vi "query Marker Frequency Count Value.vi"(8 "error in (no error)":errorcluster, 10 "Marker Index":i32=1 min=1, 11 "FSV-40N in":refnum<class "FSV-40N.lvclass">) -> (0 "error out":errorcluster, 2 "Marker Value":T1 {"X-axis" format="%#_6p"}, 3 "FSV-40N out":refnum<class "FSV-40N.lvclass">)   [LabVIEW 2023, in "Spectrum Analyzer.lvlib" / "FSV-40N.lvclass"]
uses:
  FSV-40N.lvclass
  FSV-40N.lvclass/FSV-40N.ctl
  TYPE DEFINITION/TYPE Marker Control Mode.ctl
  Spectrum Analyzer.lvlib
  <vilib>/ErrorRing/Error Ring.xnode
  TYPE DEFINITION/TYPE Marker Value.ctl
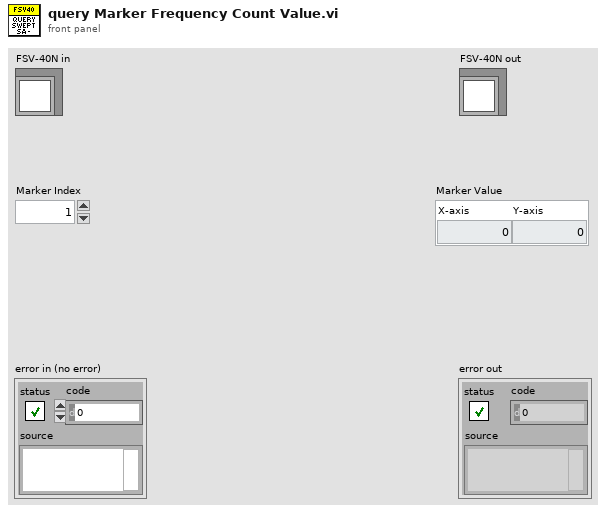
[diagram p1: front panel]
types:
  T1 = typedef "Spectrum Analyzer.lvlib/TYPE Marker Value.ctl" = cluster{"X-axis":dbl, "Y-axis":dbl}
  T2 = typedef "Spectrum Analyzer.lvlib/TYPE Marker Control Mode.ctl" = enum16{"Normal", "Delta", "Off"}
  T3 = typedef "Spectrum Analyzer.lvlib/TYPE Marker Type Map.ctl" = map{i32, T2}
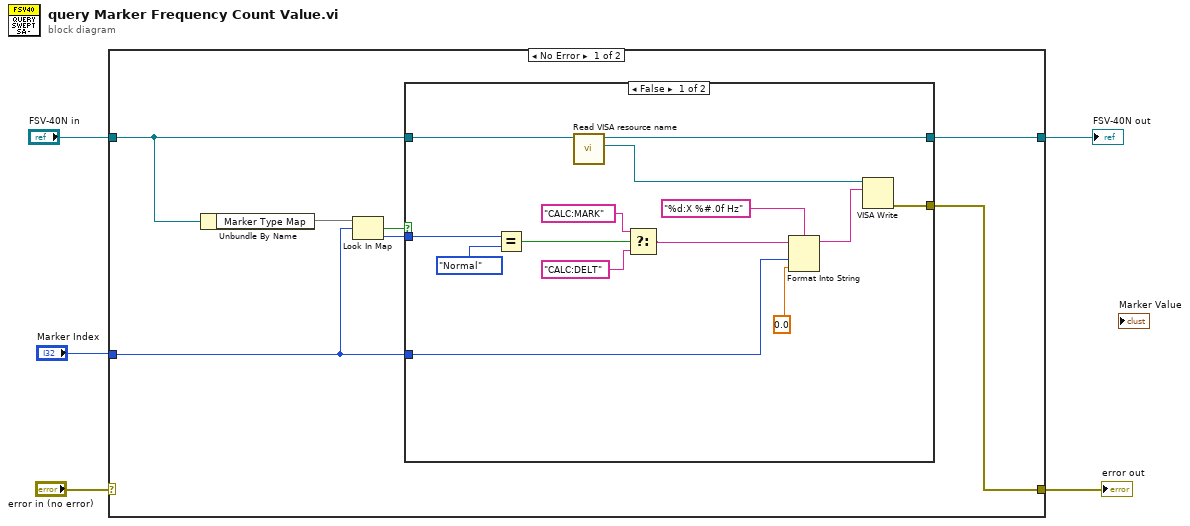
[diagram p0: block diagram]
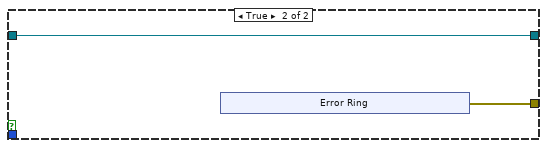
[diagram p2: hidden frame]
diagram:
  n1 = case shown="No Error" "error in (no error)" {
    selector: "error in (no error)" -> [_ w30]
    tunnel: "FSV-40N in" -> [w10 w31]
    tunnel: [w12 w31] -> w4
    tunnel: [w11 w30] -> w1
    tunnel: "Marker Index" -> [w8 _]
    frame No Error {
      n2 = Unbundle By Name(w10) -> ("Marker Type Map"=w9:T3)
      n3 = Look In Map(map=w9, key=w8) -> (key not found?=w6:bool, value=w7:T2)  [unwired: 1 in]
      n4 = case shown="False" w6 {
        tunnel: [w25 w28] -> w12
        tunnel: [w22 w27] -> w11
        tunnel: w10 -> [w21 w28]
        tunnel: w8 -> [w20 _]
        tunnel: w7 -> [w19 _]
        frame False {
          n5 = Equal?(x=w19, y=TYPE_Marker_Control_Mode."Normal") -> (x = y?=w17:bool)
          n6 = call "Read VISA resource name.vi"("FSV-40N in"=w21) -> ("VISA resource name"=w26:refnum<visa-resource-name>, "FSV-40N out"=w25:refnum<class "FSV-40N.lvclass">)  [unwired: 8 in, 1 out]
          n7 = Select(t="CALC:MARK" ("initial string"), s=w17, f="CALC:DELT" ("initial string")) -> (s? t:f=w14:string)
          n8 = Format Into String(format string="%d:X %#.0f Hz", initial string=w14, w20, 0.0 ("input 2")) -> (resulting string=w23:string)  [unwired: 1 in, 1 out]
          n9 = VISA Write(VISA resource name=w26, write buffer=w23) -> (error out=w22:errorcluster)  [unwired: 1 in, 2 out]
        }
        frame True {
          n10 = xnode "Error Ring"() -> ("error out"=w27:errorcluster)
        }
      }
    }
    frame Error {
    }
  }
  "error out" <- w1
  "FSV-40N out" <- w4
